vi "lvmcp_constvalue.vi"() -> ()   [LabVIEW 2026]
panel:
  out "error out":errorcluster
  in  "data string":string
  in  "type string":string
  in  "reference":refnum<vi>
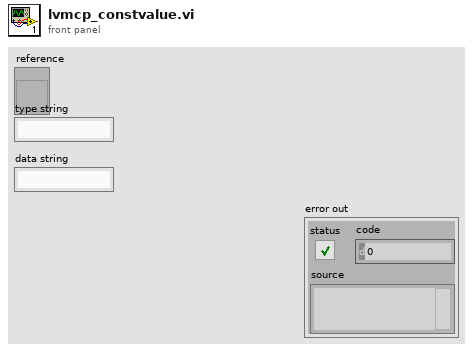
[diagram p1: front panel]
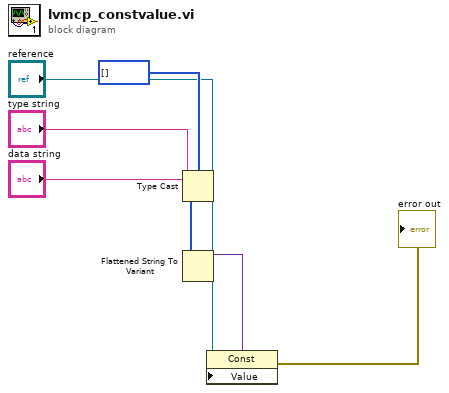
[diagram p0: block diagram]
diagram:
  n1 = Type Cast(type=i16[] [], x="type string") -> (*(type *) &x=w6:i16[])
  n2 = Flattened String To Variant(6:"data string", 7:w6) -> (0:w2:errorcluster, 3:w4:variant)  [unwired: 1 in]
  n3 = property class="Const"(reference="reference", error in=w2, "Value"=w4) -> (error out=→"error out":errorcluster)  [unwired: 1 out]
